vi "Register OK Notifier Name.vi"() -> (0 "register ok notifier":string)   [LabVIEW 2018, in "GLog.lvlib" / "UI Updater.lvlib"]
uses:
  UI Updater.lvlib
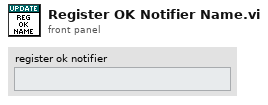
[diagram p1: front panel]
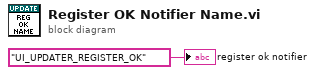
[diagram p0: block diagram]
diagram:
  "register ok notifier" <- "UI_UPDATER_REGISTER_OK" ("name (unnamed)")
